vi "Wait on Ready for Events Notification.vi"(8 "error in (no error)":errorcluster, 11 "timeout [ms]":i32) -> (0 "error out":errorcluster)   [LabVIEW 2018, in "GLog.lvlib" / "Registry.lvlib"]
uses:
  Registry.lvlib
  <vilib>/Utility/error.llb/Error Cluster From Error Code.vi
  <vilib>/ErrorRing/Error Ring.xnode
panel:
  # "Connector Pane"
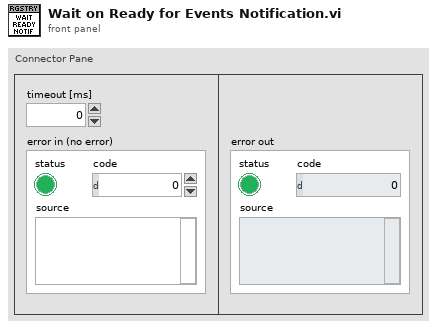
[diagram p1: front panel]
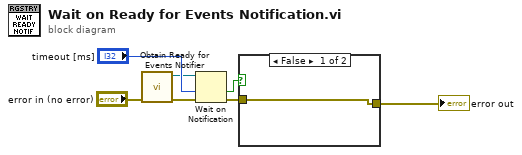
[diagram p0: block diagram]
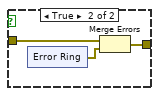
[diagram p2: hidden frame]
diagram:
  n1 = call "Obtain Ready for Events Notifier.vi"("error in (no error)"="error in (no error)") -> ("error out"=w2:errorcluster, "notifier"=w4:refnum<notifier>)  [unwired: 9 in]
  n2 = Wait on Notification(notifier=w4, timeout in ms (-1)="timeout [ms]", error in (no error)=w2) -> (timed out?=w7:bool, error out=w6:errorcluster)  [unwired: 1 in, 2 out]
  n3 = case shown="False" w7 {
    tunnel: w6 -> [w8 w11]
    tunnel: [w8 w9] -> w3
    frame False {
    }
    frame True {
      n4 = xnode "Error Ring"() -> ("error out"=w10:errorcluster)
      n5 = Merge Errors(w11, w10) -> (w9:errorcluster)
    }
  }
  "error out" <- w3
